vi "VIH ProjFile - Item Rule Array - Write.vi"(7 "Project Folder":path, 8 "error in":errorcluster, 9 "Item Rules":T1[](array[typedef]), 10 "Item Paths":path[](array[path]), 11 "XML Parent Item":refnum<k20>) -> (0 "error out":errorcluster, 3 "dup XML Parent Item":refnum<k20>)   [LabVIEW 2014]
doc: "::: VI Helpeks :::\nCopyright (c) 2000-2026 Konstantin Shifershteyn. All rights reserved."
uses:
  _VIH HelpGen.llb/VIH HelpGen Typedef - Cluster - File Rule.ctl
  _VIH HelpGen.llb/VIH HelpGen Typedef - Enum - Default,Enable,Disable.ctl
  _VIH HelpGen.llb/VIH HelpGen Typedef - Cluster - File Rule - Source Paths.ctl
  _VIH HelpGen.llb/VIH HelpGen Typedef - Cluster - File Rule - Target Paths.ctl
  _VIH HelpGen.llb/VIH HelpGen Typedef - Enum - Description Mode.ctl
  _VIH HelpGen.llb/VIH HelpGen Typedef - Cluster - Control Rule.ctl
  _VIH HelpGen.llb/VIH HelpGen Typedef - Cluster - Enum Value Info.ctl
  _VIH HelpGen.llb/VIH HelpGen Typedef - Cluster - Group Rule - Flags.ctl
  <vilib>/xml/Close Reference(Node).vi
  <resource>/objmgr/DOMUserDefRef.rc
  <vilib>/xml/NI_XML.lvlib
panel:
  # "VI Helpeks\nCopyright (c) 2012-2026 Konstantin Shifershteyn"
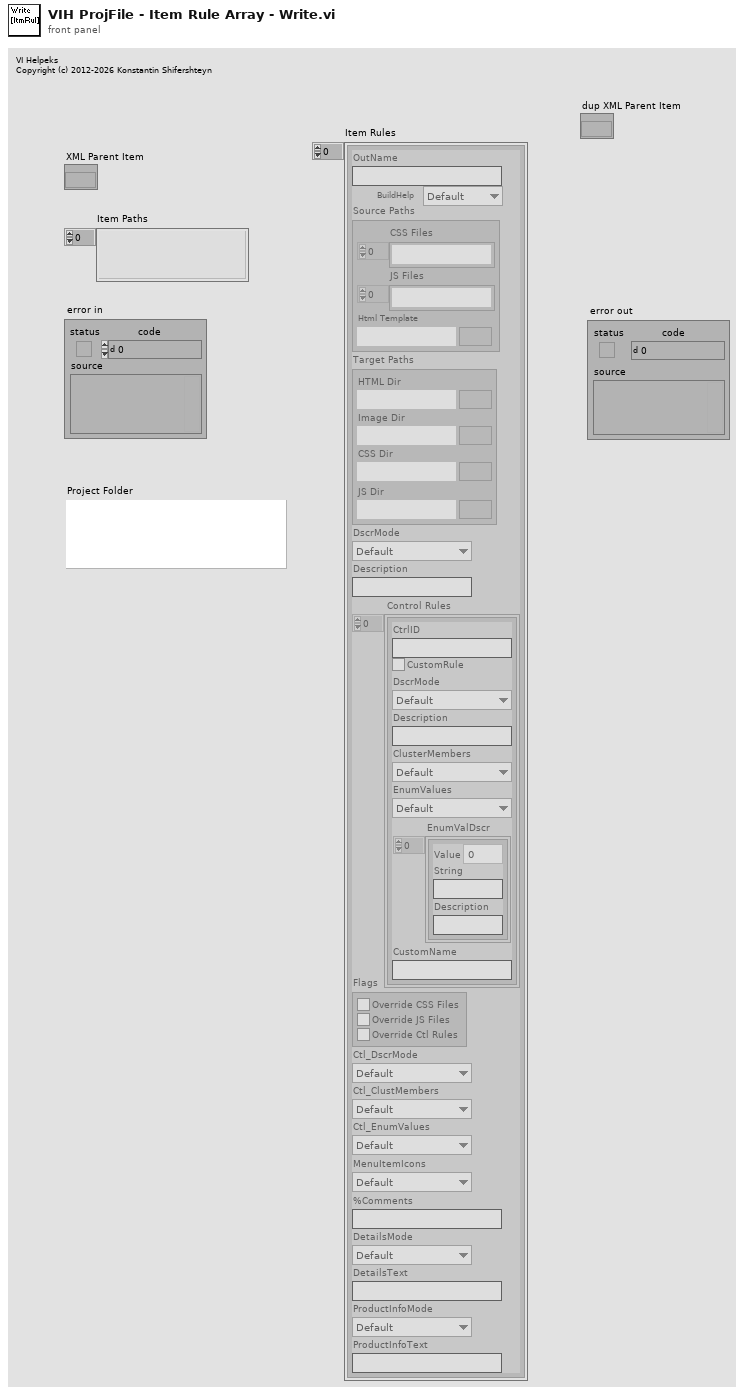
[diagram p1: front panel]
types:
  T1 = typedef "VIH HelpGen Typedef - Cluster - File Rule.ctl" = cluster{"OutName":string, "BuildHelp":T2, "Source Paths":T3, "Target Paths":T4, "DscrMode":T5, "Description":string, "Control Rules":T6[], "Flags":T8, "Ctl_DscrMode":T5, "Ctl_ClustMembers":T2, "Ctl_EnumValues":T2, "MenuItemIcons":T2, "%Comments":string, "DetailsMode":T5, "DetailsText":string, "ProductInfoMode":T2, "ProductInfoText":string}
  T2 = typedef "VIH HelpGen Typedef - Enum - Default,Enable,Disable.ctl" = enum16{"Default", "Enable", "Disable"}
  T3 = typedef "VIH HelpGen Typedef - Cluster - File Rule - Source Paths.ctl" = cluster{"CSS Files":path[], "JS Files":path[], "Html Template":path}
  T4 = typedef "VIH HelpGen Typedef - Cluster - File Rule - Target Paths.ctl" = cluster{"HTML Dir":path, "Image Dir":path, "CSS Dir":path, "JS Dir":path}
  T5 = typedef "VIH HelpGen Typedef - Enum - Description Mode.ctl" = enum16{"Default", "Description", "Description1", "Description2", "Custom", "None"}
  T6 = typedef "VIH HelpGen Typedef - Cluster - Control Rule.ctl" = cluster{"CtrlID":string, "CustomRule":bool, "DscrMode":T5, "Description":string, "ClusterMembers":T2, "EnumValues":T2, "EnumValDscr":T7[], "CustomName":string}
  T7 = typedef "VIH HelpGen Typedef - Cluster - Enum Value Info.ctl" = cluster{"Value":ext, "String":string, "Description":string}
  T8 = typedef "VIH HelpGen Typedef - Cluster - Group Rule - Flags.ctl" = cluster{"Override CSS Files":bool, "Override JS Files":bool, "Override Ctl Rules":bool}
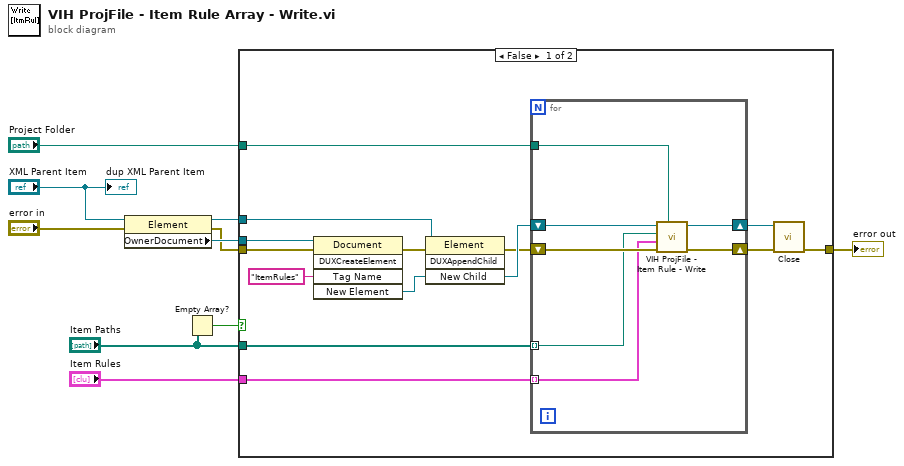
[diagram p0: block diagram]
diagram:
  n1 = property class="Element"(reference="XML Parent Item", error in="error in") -> (reference out=w4:refnum<k20>, error out=w3:errorcluster, "OwnerDocument"=w5:refnum<k20>)
  n2 = Empty Array?(array="Item Paths") -> (empty?=w10:bool)
  n3 = case shown="False" w10 {
    tunnel: w4 -> [w23 _]
    tunnel: w3 -> [w22 w31]
    tunnel: [w15 w31] -> w9
    tunnel: "Item Paths" -> [w14 _]
    tunnel: "Item Rules" -> [w13 _]
    tunnel: w5 -> [w12 _]
    tunnel: "Project Folder" -> [w11 _]
    frame False {
      n4 = invoke class="Document" method="DUXCreateElement"(reference=w12, error in=w22, "Tag Name"="ItemRules") -> (error out=w20:errorcluster, "New Element"=w19:refnum<k20>)  [unwired: 2 in, 3 out]
      n5 = invoke class="Element" method="DUXAppendChild"(reference=w23, error in=w20, "New Child"=w19) -> (error out=w18:errorcluster)  [unwired: 1 in, 3 out]
      n6 = for {
        shift-right: [w29] -> w16
        shift-left: w18 -> [w30]
        shift-right: [w25] -> w17
        shift-left: w19 -> [w27]
        tunnel: w14 -> [w28] mode=indexing
        tunnel: w13 -> [w26] mode=indexing
        tunnel: w11 -> [w24]
        n7 = call "VIH ProjFile - Item Rule - Write.vi"("Project Folder"=w24, "error in"=w30, "Item Rule"=w26, "Path"=w28, "XML Parent Item"=w27) -> ("error out"=w29:errorcluster, "dup XML Parent Item"=w25:refnum<k20>)  [unwired: 5 in]
      }
      n8 = call-poly <vilib>:"Close.vi"("error in (no error)"=w16, "node"=w17) -> ("error out"=w15:errorcluster)  [unwired: 7 in]
    }
    frame True {
    }
  }
  "error out" <- w9
  "dup XML Parent Item" <- "XML Parent Item"
